vi "JSON to Status Tree.vi"(9 "JSON":string, 10 "Status Tree in":map{string[], T1}(c390)) -> (0 "error out":errorcluster, 2 "Status Tree":map{string[], T1}(c390))   [LabVIEW 2020, in "Volatus.lvlib" / "DebugHTTPController.lvclass"]
uses:
  DebugHTTPController.lvclass
  Module Status.ctl
  Module/State.ctl
  lv-cdm/CDM-Config/Config Element/Config Element.lvclass
  DebugHTTPController.lvclass/DebugHTTPController.ctl
  lv-cdm/CDM-Config/Config-JSON/Config-JSON.lvclass
  Module/Module.lvclass
  Volatus.lvlib
  lv-cdm/CDM-Config/Config Manager/Config Manager.lvclass
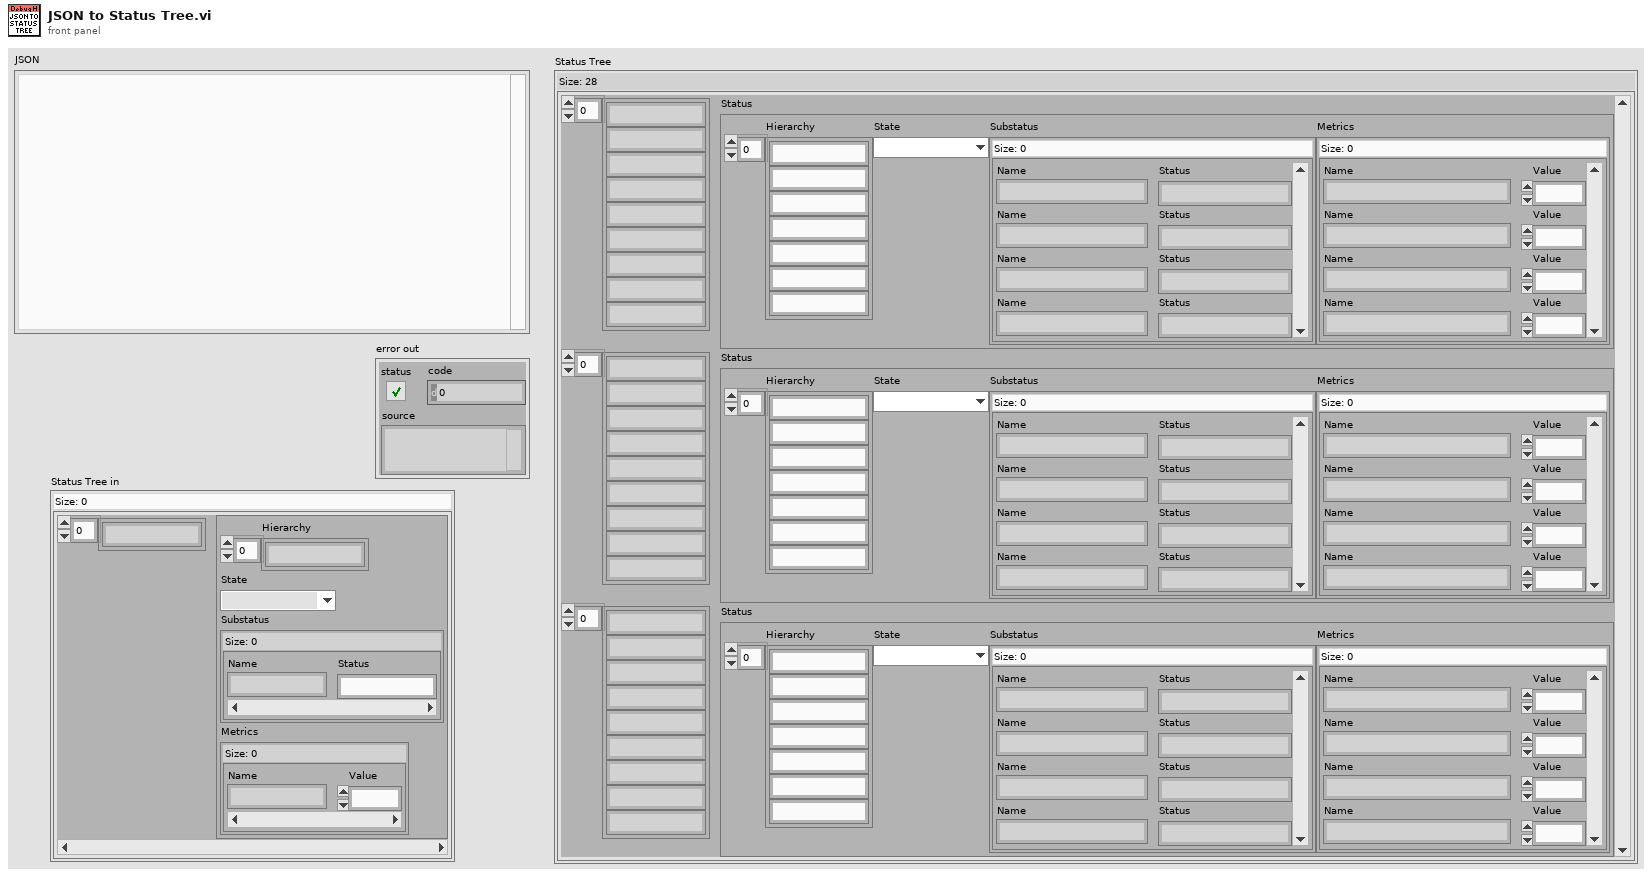
[diagram p1: front panel]
types:
  T1 = typedef "Volatus.lvlib/Module Status.ctl" = cluster{"Hierarchy":string[], "State":T2, "Substatus":map{string, string}, "Metrics":map{string, dbl}}
  T2 = typedef "Volatus.lvlib/Module.lvclass/State.ctl" = enum16{"Unknown", "Launched", "Starting", "Running", "Stopping", "Stopped", "Error - Starting", "Error - Run", "Error - Stopping"}
  T3 = cluster{"Parent":string[], "Element":refnum<class "Config Element.lvclass">}
  T4 = cluster{"Parent":string[], "Elements":refnum<class "Config Element.lvclass">}
  T5 = cluster{string[], "Elements":refnum<class "Config Element.lvclass">}
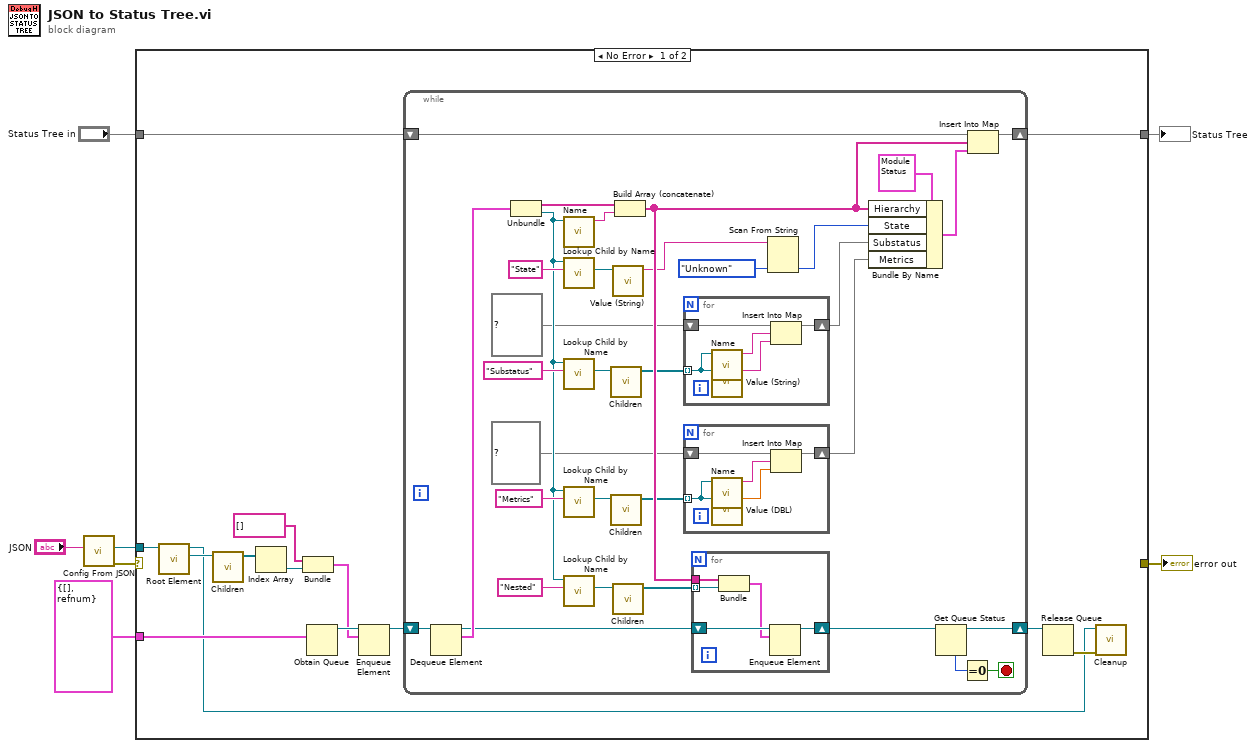
[diagram p0: block diagram]
diagram:
  n1 = call "Config From JSON.vi"("JSON"="JSON") -> ("error out"=w6:errorcluster, "Config"=w5:refnum<class "Config Manager.lvclass">)  [unwired: 9 in]
  n2 = case shown="No Error" w6 {
    selector: w6 -> [_ w71]
    tunnel: w5 -> [w21 _]
    tunnel: T3 {"Parent"=[], "Element"=refnum} -> [w18 _]
    tunnel: [w12 w70] -> w3
    tunnel: [_ w71] -> w2
    tunnel: "Status Tree in" -> [w8 w70]
    frame No Error {
      n3 = call "Root Element.vi"("Config Manager in"=w21) -> ("Root Element"=w20:refnum<class "Config Element.lvclass">, "Config Manager out"=w9:refnum<class "Config Manager.lvclass">)  [unwired: 8 in, 1 out]
      n4 = call "Children.vi"("Config Element in"=w20) -> ("Elements"=w19:refnum<class "Config Element.lvclass">[])  [unwired: 9 in, 1 out]
      n5 = Index Array(array=w19) -> (element=w16:refnum<class "Config Element.lvclass">)  [unwired: 1 in]
      n6 = Bundle("Parent"=string[] [], "Elements"=w16) -> (w15:T4)  [unwired: 1 in]
      n7 = Obtain Queue(element data type=w18) -> (queue out=w17:refnum<queue>)  [unwired: 4 in, 2 out]
      n8 = Enqueue Element(queue=w17, element=w15) -> (queue out=w13:refnum<queue>)  [unwired: 2 in, 2 out]
      n9 = while {
        shift-right: [w49] -> w11
        shift-left: w13 -> [w54]
        shift-right: [w44] -> w12
        shift-left: w8 -> [w46]
        stop <- w47 stop-if-true
        n10 = Dequeue Element(queue=w54) -> (queue out=w37:refnum<queue>, element=w53:T3)  [unwired: 2 in, 2 out]
        n11 = Unbundle(w53) -> ("Parent"=w52:string[], "Element"=w39:refnum<class "Config Element.lvclass">)
        n12 = call "Name.vi"("Config Element in"=w39) -> ("Name"=w51:string)  [unwired: 9 in, 1 out]
        n13 = call "Lookup Child by Name.vi"("Name"="State", "Config Element in"=w39) -> ("Child"=w28:refnum<class "Config Element.lvclass">)  [unwired: 6 in, 3 out]
        n14 = call "Lookup Child by Name.vi"("Name"="Substatus", "Config Element in"=w39) -> ("Child"=w33:refnum<class "Config Element.lvclass">)  [unwired: 6 in, 3 out]
        n15 = call "Lookup Child by Name.vi"("Name"="Metrics", "Config Element in"=w39) -> ("Child"=w32:refnum<class "Config Element.lvclass">)  [unwired: 6 in, 3 out]
        n16 = call "Lookup Child by Name.vi"("Name"="Nested", "Config Element in"=w39) -> ("Child"=w38:refnum<class "Config Element.lvclass">)  [unwired: 6 in, 3 out]
        n17 = call "Children.vi"("Config Element in"=w33) -> ("Elements"=w31:refnum<class "Config Element.lvclass">[])  [unwired: 9 in, 1 out]
        n18 = call "Children.vi"("Config Element in"=w32) -> ("Elements"=w24:refnum<class "Config Element.lvclass">[])  [unwired: 9 in, 1 out]
        n19 = call "Value (String).vi"("Config Element in"=w28) -> ("String Value"=w22:string)  [unwired: 9 in, 1 out]
        n20 = call "Children.vi"("Config Element in"=w38) -> ("Elements"=w36:refnum<class "Config Element.lvclass">[])  [unwired: 9 in, 1 out]
        n21 = Build Array (concatenate)(w52, w51) -> (w35:string[])
        n22 = for {
          tunnel: w31 -> [w64] mode=indexing
          shift-right: [w60] -> w29
          shift-left: map{string, string} {} ("Substatus") -> [w63]
          n23 = call "Name.vi"("Config Element in"=w64) -> ("Name"=w62:string)  [unwired: 9 in, 1 out]
          n24 = call "Value (String).vi"("Config Element in"=w64) -> ("String Value"=w61:string)  [unwired: 9 in, 1 out]
          n25 = Insert Into Map(map in=w63, key=w62, value=w61) -> (map out=w60:map{string, string})  [unwired: 2 out]
        }
        n26 = for {
          tunnel: w24 -> [w59] mode=indexing
          shift-right: [w55] -> w23
          shift-left: map{string, dbl} {} ("Metrics") -> [w58]
          n27 = call "Name.vi"("Config Element in"=w59) -> ("Name"=w57:string)  [unwired: 9 in, 1 out]
          n28 = call "Value (DBL).vi"("Config Element in"=w59) -> ("DBL Value"=w56:dbl)  [unwired: 9 in, 1 out]
          n29 = Insert Into Map(map in=w58, key=w57, value=w56) -> (map out=w55:map{string, dbl})  [unwired: 2 out]
        }
        n30 = for {
          shift-right: [w65] -> w34
          shift-left: w37 -> [w67]
          tunnel: w36 -> [w69] mode=indexing
          tunnel: w35 -> [w68]
          n31 = Bundle(w68, "Elements"=w69) -> (w66:T5)  [unwired: 1 in]
          n32 = Enqueue Element(queue=w67, element=w66) -> (queue out=w65:refnum<queue>)  [unwired: 2 in, 2 out]
        }
        n33 = Scan From String(input string=w22, default 1=State."Unknown" ("State")) -> (output 1=w26:T2)  [unwired: 3 in, 3 out]
        n34 = Bundle By Name(cluster=T1 {"Hierarchy"=[], "State"=enum."Unknown", "Substatus"={}, "Metrics"={}} ("Module Status"), "Hierarchy"=w35, "State"=w26, "Substatus"=w29, "Metrics"=w23) -> (w45:T1)
        n35 = Get Queue Status(queue=w34) -> (queue out=w49:refnum<queue>, # elements in queue=w48:i32)  [unwired: 2 in, 6 out]
        n36 = Equal To 0?(x=w48) -> (x = 0?=w47:bool)
        n37 = Insert Into Map(map in=w46, key=w35, value=w45) -> (map out=w44:map{string[], T1})  [unwired: 2 out]
      }
      n38 = Release Queue(queue=w11) -> (error out=w10:errorcluster)  [unwired: 2 in, 2 out]
      n39 = call "Cleanup.vi"("error in (no error)"=w10, "Config Manager in"=w9) -> ()  [unwired: 9 in, 1 out]
    }
    frame Error {
    }
  }
  "Status Tree" <- w3
  "error out" <- w2
